vi "VIH - VI Doc Editor - Shortcut Menu Handler - Tree.vi"(6 "Menu Tag":string, 9 "MenuRef":refnum<k9>, 10 "Terminals Tree":refnum<vi>, 11 "Event Type":T1) -> (3 "States spec":string)   [LabVIEW 2014]
doc: "::: VI Helpeks :::\nCopyright (c) 2000-2026 Konstantin Shifershteyn. All rights reserved."
uses:
  <vilib>/event_ctls.llb/lveventtype.ctl
  <vilib>/Utility/miscctls.llb/LVNodeAndColumnTypeDef.ctl
  _VIH Support Library.llb/VIH Utility - MENU - Create Menu (String).vi
panel:
  # "VI Helpeks\nCopyright (c) 2012-2026 Konstantin Shifershteyn"
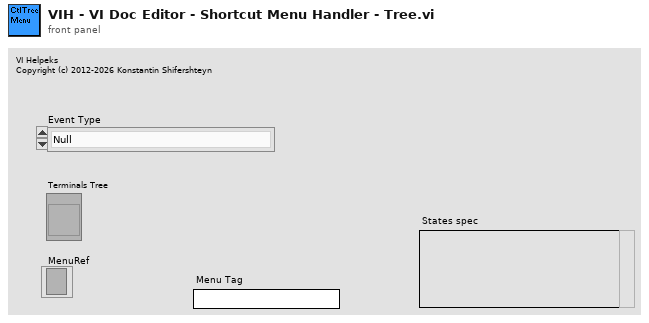
[diagram p1: front panel]
types:
  T1 = typedef "lveventtype.ctl" = enum32{"Null", "Timeout", "Annotation Menu Selection", "Annotation Menu Selection?", "App Instance Close", "App Instance Close?", "Autoscale Range Change", "Bookmark Info Change", "Cell Edit", "Cell Edit?", "Cursor Grab", "Cursor Grab?", "Cursor Menu Selection", "Cursor Menu Selection?", "Cursor Move", "Cursor Release", "Data Change", "Direction Change", "Display State Change", "Drag Ended", "Drag Enter", "Drag Leave", "Drag Over", "Drag Source Update", "Drag Starting", "Drag Starting?", "Drop", "Exec State Change", "Key Down", "Key Down?", "Key Repeat", "Key Repeat?", "Key Up", "Listbox Double Click", "Menu Activation?", "Menu Selection (App)", "Menu Selection? (App)", "Menu Selection (User)", "Mouse Down", "Mouse Down?", "Mouse Enter", "Mouse Leave", "Mouse Move", "Mouse Up", "Mouse Wheel", "NI Security User Change (App)", "Pane Size", "Panel Close", "Panel Close?", "Panel Resize", "Plot Attribute Change", "Scale Range Change", "Shortcut Menu Activation?", "Shortcut Menu Selection (App)", "Shortcut Menu Selection? (App)", "Shortcut Menu Selection (User)", "Tree Double Click", "Tree Drag", "Tree Drag?", "Tree Drop", "Tree Drop?", "Tree Item Close", "Tree Item Close?", "Tree Item Open", "Tree Item Open?", "User Event", "Value Change"}
  T2 = typedef "LVNodeAndColumnTypeDef.ctl" = cluster{"Node":string, "Column":i32}
  T3 = typedef "VIH Project Tree Typedef - Tree Refnum.ctl" = refnum<vi>
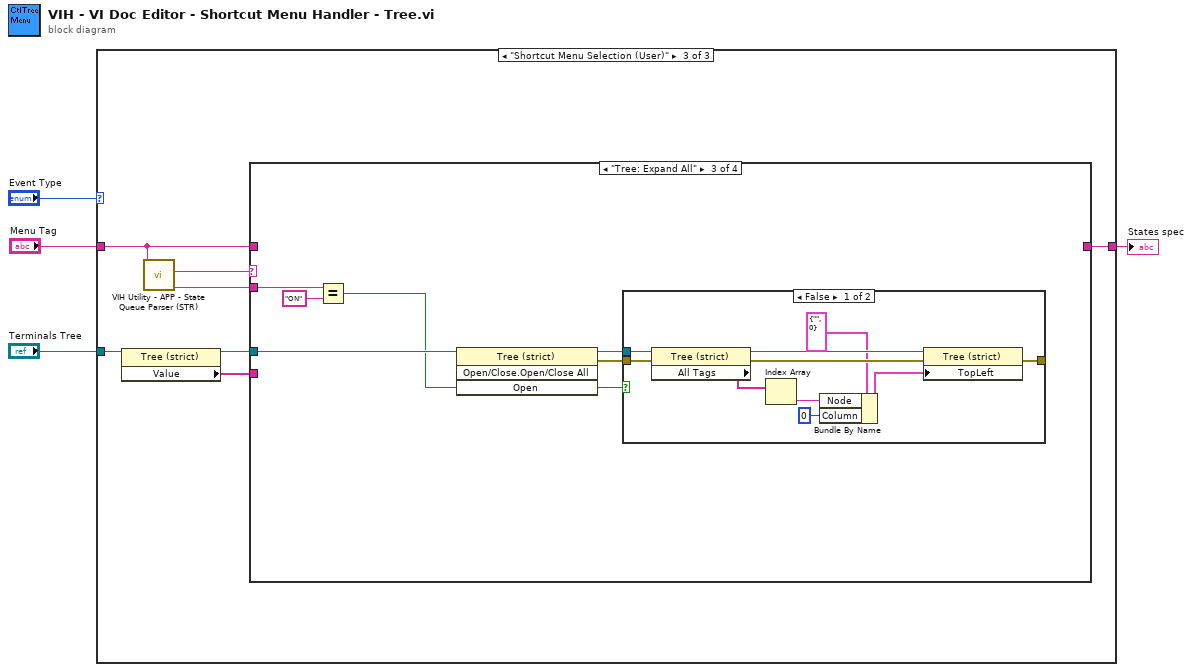
[diagram p0: block diagram]
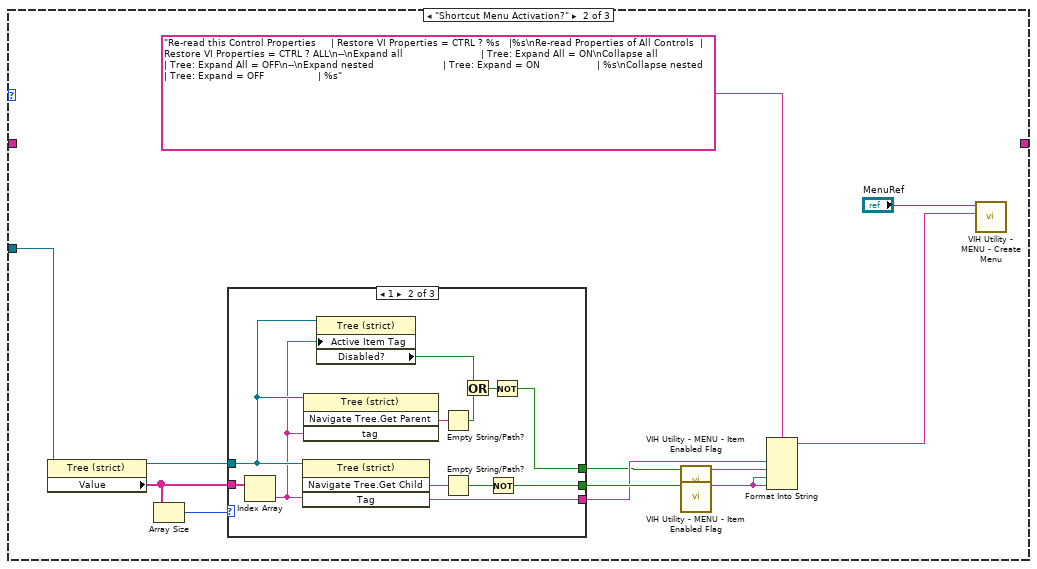
[diagram p3: hidden frame]
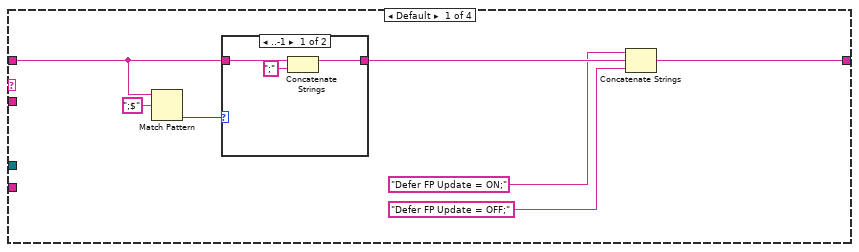
[diagram p6: hidden frame]
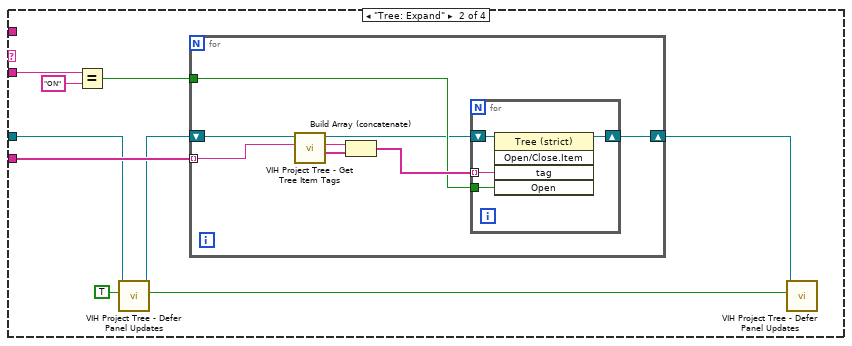
[diagram p8: hidden frame]
diagram:
  n1 = case shown="\"Shortcut Menu Selection (User)\"" "Event Type" {
    tunnel: "Terminals Tree" -> [_ w16 w31]
    tunnel: [_ _ w29] -> w2
    tunnel: "Menu Tag" -> [_ _ w33]
    frame Default {
    }
    frame "Shortcut Menu Activation?" {
      n2 = property class="Tree (strict)"(reference=w16) -> (reference out=w13:refnum<vi>, "Value"=w8:string[])  [unwired: 1 in, 1 out]
      n3 = Array Size(array=w8) -> (size(s)=w10:i32)
      n4 = case shown="1" w10 {
        tunnel: w13 -> [_ w21 _]
        tunnel: [_ w25 _] -> w9
        tunnel: w8 -> [_ w24 _]
        tunnel: [_ w20 _] -> w7
        tunnel: [_ w22 _] -> w6
        frame ..0 {
        }
        frame 1 {
          n5 = Index Array(array=w24) -> (element=w20:string)  [unwired: 1 in]
          n6 = invoke class="Tree (strict)" method="Navigate Tree.Get Child"(reference=w21, "Tag"=w20) -> ("Navigate Tree:Get Child"=w27:string)  [unwired: 2 in, 3 out]
          n7 = invoke class="Tree (strict)" method="Navigate Tree.Get Parent"(reference=w21, "tag"=w20) -> ("Navigate Tree:Get Parent"=w23:string)  [unwired: 2 in, 3 out]
          n8 = property class="Tree (strict)"(reference=w21, "Active Item Tag"=w20) -> ("Disabled?"=w19:bool)  [unwired: 1 in, 2 out]
          n9 = Empty String/Path?(string/path=w23) -> (empty?=w18:bool)
          n10 = Empty String/Path?(string/path=w27) -> (empty?=w26:bool)
          n11 = Or(x=w19, y=w18) -> (x .or. y?=w17:bool)
          n12 = Not(x=w26) -> (.not. x?=w25:bool)
          n13 = Not(x=w17) -> (.not. x?=w22:bool)
        }
        frame 2.. {
        }
      }
      n14 = call "VIH Utility - MENU - Item Enabled Flag.vi"("Enable?"=w6) -> ("Disable flag"=w5:string)  [unwired: 10 in]
      n15 = call "VIH Utility - MENU - Item Enabled Flag.vi"("Enable?"=w9) -> ("Disable flag"=w11:string)  [unwired: 10 in]
      n16 = Format Into String(format string="Re-read this Control Properties     | Restore VI Properties = CTRL ? %s   |%s\nRe-read Properties of All Controls  | Restore VI Properties = CTRL ? ALL\n--\nExpand all                          | Tree: Expand All = ON\nCollapse all                        | Tree: Expand All = OFF\n--\nExpand nested                       | Tree: Expand = ON                   | %s\nCollapse nested                     | Tree: Expand = OFF                  | %s", w7, w5, w11, w11) -> (resulting string=w12:string)  [unwired: 2 in, 1 out]
      n17 = call-poly "VIH Utility - MENU - Create Menu.vi"("Menu Description"=w12, "menu"="MenuRef") -> ()  [unwired: 8 in, 2 out]
    }
    frame "Shortcut Menu Selection (User)" {
      n18 = property class="Tree (strict)"(reference=w31) -> (reference out=w30:refnum<vi>, "Value"=w32:string[])  [unwired: 1 in, 1 out]
      n19 = call "VIH Utility - APP - State Queue Parser (STR).vi"("input queue"=w33) -> ("state parameters"=w28:string, "state"=w34:string)  [unwired: 5 in, 2 out]
      n20 = case shown="\"Tree: Expand All\"" w34 {
        tunnel: [w37 _ _ _] -> w29
        tunnel: w33 -> [w39 _ _ _]
        tunnel: w30 -> [_ w51 w70 _]
        tunnel: w32 -> [_ w54 _ _]
        tunnel: w28 -> [_ w53 w72 _]
        frame Default {
          n21 = Match Pattern(string=w39, regular expression=";$") -> (offset past match=w40:i32)  [unwired: 1 in, 3 out]
          n22 = case shown="..-1" w40 {
            tunnel: w39 -> [w44 w45]
            tunnel: [w43 w45] -> w38
            frame ..-1 {
              n23 = Concatenate Strings(w44, ";" ("string")) -> (w43:string)
            }
            frame 0.. {
            }
          }
          n24 = Concatenate Strings("Defer FP Update = ON;", w38, "Defer FP Update = OFF;") -> (w37:string)
        }
        frame "Tree: Expand" {
          n25 = Equal?(x=w53, y="ON") -> (x = y?=w46:bool)
          n26 = call "VIH Project Tree - Defer Panel Updates.vi"("Defer Panel Updates (F)"=TRUE, "Project Tree"=w51) -> ("Previous Defer status"=w48:bool, "dup Project Tree"=w50:T3)  [unwired: 7 in, 1 out]
          n27 = for {
            tunnel: w54 -> [w59] mode=indexing
            shift-right: [w60] -> w49
            shift-left: w50 -> [w62]
            tunnel: w46 -> [w56]
            n28 = call "VIH Project Tree - Get Tree Item Tags.vi"("Parent Item Tag"=w59, "Project Tree"=w62) -> ("Child Item Tags"=w57:string[], "dup Parent Item Tag"=w58:string, "dup Project Tree"=w55:T3)  [unwired: 6 in, 1 out]
            n29 = Build Array (concatenate)(w58, w57) -> (w61:string[])
            n30 = for {
              tunnel: w61 -> [w65] mode=indexing
              tunnel: w56 -> [w64]
              shift-right: [w63] -> w60
              shift-left: w55 -> [w66]
              n31 = invoke class="Tree (strict)" method="Open/Close.Item"(reference=w66, "tag"=w65, "Open"=w64) -> (reference out=w63:T3)  [unwired: 2 in, 4 out]
            }
          }
          n32 = call "VIH Project Tree - Defer Panel Updates.vi"("Defer Panel Updates (F)"=w48, "Project Tree"=w49) -> ()  [unwired: 7 in, 3 out]
        }
        frame "Tree: Expand All" {
          n33 = Equal?(x=w72, y="ON") -> (x = y?=w67:bool)
          n34 = invoke class="Tree (strict)" method="Open/Close.Open/Close All"(reference=w70, "Open"=w67) -> (reference out=w69:refnum<vi>, error out=w68:errorcluster)  [unwired: 2 in, 2 out]
          n35 = case shown="False" w67 {
            tunnel: [w79 w83] -> _
            tunnel: w68 -> [w77 w83]
            tunnel: w69 -> [w76 _]
            frame False {
              n36 = property class="Tree (strict)"(reference=w76, error in=w77) -> (reference out=w75:refnum<vi>, error out=w78:errorcluster, "All Tags"=w82:string[])
              n37 = Index Array(array=w82) -> (element=w81:string)  [unwired: 1 in]
              n38 = Bundle By Name(cluster=T2 {"Node"="", "Column"=0} ("Top Left Visible Cell"), "Node"=w81, "Column"=0) -> (w73:T2)
              n39 = property class="Tree (strict)"(reference=w75, error in=w78, "TopLeft"=w73) -> (error out=w79:errorcluster)  [unwired: 1 out]
            }
            frame True {
            }
          }
        }
        frame "----------------------------- 1" {
        }
      }
    }
  }
  "States spec" <- w2
